vi "Panel.vi"(11 "SequenceViewPanel in":refnum<class "SequenceViewPanel.lvclass">) -> ()   [LabVIEW 2020, in "TSnax UI.lvlib" / "SequenceViewPanel.lvclass"]
uses:
  SequenceViewPanel.lvclass
  C:/Program Files (x86)/National Instruments/LabVIEW 2020/vi.lib/IlluminatedG/IG OOPanel/OOPanel/Panel/Panel.lvclass
  <vilib>/IlluminatedG/IG OOPanel/OOPanel/Panel/Basic UI State.ctl
  <vilib>/IlluminatedG/IG OOPanel/OOPanel/Panel/Panel Events.ctl
  <vilib>/IlluminatedG/IG OOPanel/OOPanel/Panel/Visbility Event Data.ctl
  <vilib>/IlluminatedG/IG OOPanel/OOPanel/Panel/Visibility State.ctl
  <vilib>/IlluminatedG/IG OOPanel/OOPanel/Panel/Close Reason.ctl
  Incoming Events.ctl
  Set SequenceFile Request.ctl
  TSnax/SequenceFile/SequenceFile.lvclass
  C:/dev/illuminated-g/tsnax/TSnax/PropertyObject/PropertyObject.lvclass
  Set SequenceFile Response.ctl
  Refresh Step Request.ctl
  TSnax/Step/Step.lvclass
  Error Response.ctl
  Step Result Request.ctl
  SequenceViewPanel.lvclass/SequenceViewPanel.ctl
  TSnax/PropertyObject/PropertyObject.lvclass/PropertyObject.ctl
  Mark Trace Data.ctl
  Trace Marker.ctl
  TSnax/Step Group.ctl
  TSnax/PropertyObject/PropertyObject Ref.vi
  UIMsg Callback.vi
  TSnax/PropertyObject/PropertyObject.lvclass
  TSnax/Sequence/Sequence.lvclass
  <vilib>/IlluminatedG/IG OOPanel/OOPanel/Panel/Panel.lvclass
  <vilib>/IlluminatedG/IG OOPanel/OOPanel/OOPanel.lvlib
  TSnax UI.lvlib
  TSnax/TSnax.lvlib
  TSnax/Engine/Engine.lvclass
  C:/dev/illuminated-g/tsnax/TSnax UI/SequenceViewPanel/SequenceViewPanel.lvclass
  C:/dev/illuminated-g/tsnax/TSnax/PropertyObjectFile/PropertyObjectFile.lvclass
  C:/dev/illuminated-g/tsnax/TSnax/SequenceFile/SequenceFile.lvclass
  TSnax/UIMessage/UIMessage.lvclass
panel:
  out "Markers":picture
  in  "Steps":string(tree)
  in  "Sequences":string(tree)
  in  "Variables":string(tree)
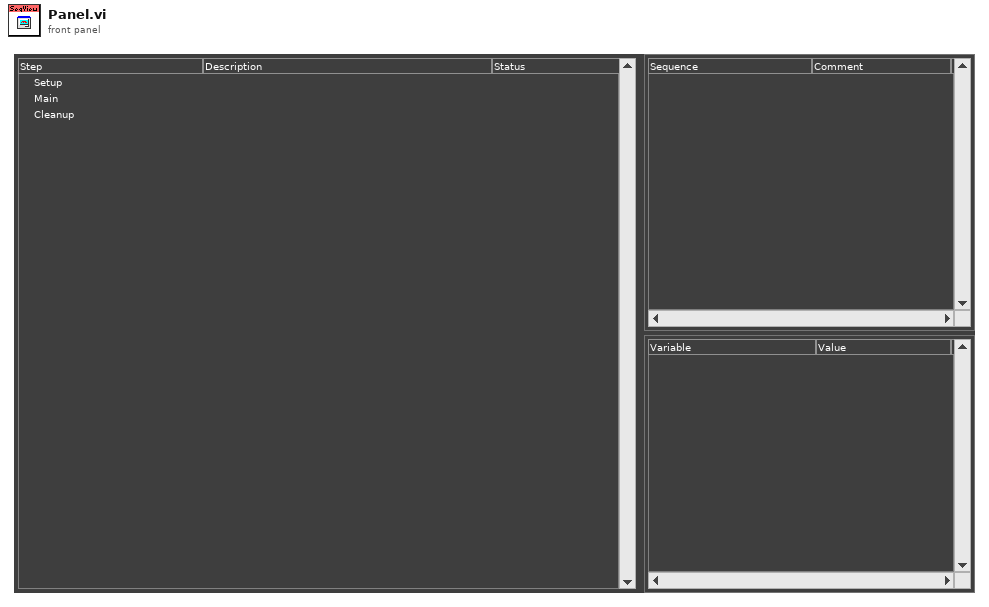
[diagram p1: front panel]
types:
  T1 = typedef "OOPanel.lvlib/Panel.lvclass/Basic UI State.ctl" = enum16{"Init", "Run", "Close"}
  T2 = typedef "TSnax UI.lvlib/SequenceViewPanel.lvclass/Set SequenceFile Response.ctl" = cluster{"Error":errorcluster}
  T3 = typedef "TSnax UI.lvlib/SequenceViewPanel.lvclass/Set SequenceFile Request.ctl" = cluster{"SequenceFile":refnum<class "SequenceFile.lvclass">, "Notifier":refnum<notifier>, "SequenceIndex":i32}
  T4 = typedef "TSnax UI.lvlib/SequenceViewPanel.lvclass/Mark Trace Data.ctl" = cluster{"Trace Marker":T5}
  T5 = typedef "TSnax UI.lvlib/SequenceViewPanel.lvclass/Trace Marker.ctl" = cluster{"TSnax:SequenceFile":refnum<class "SequenceFile.lvclass">, "SequenceIndex":i32, "StepGroup":i32, "PreviousStepIndex":i32, "NextStepIndex":i32}
  T6 = typedef "TSnax UI.lvlib/Error Response.ctl" = cluster{"Error":errorcluster}
  T7 = typedef "TSnax.lvlib/Step Group.ctl" = enum16{"Setup", "Main", "Cleanup"}
  T8 = typedef "TSnax UI.lvlib/SequenceViewPanel.lvclass/Incoming Events.ctl" = cluster{"Set SequenceFile":refnum<user-event>, "Show Sequence":refnum<user-event>, "Refresh Step":refnum<user-event>, "Step Result":refnum<user-event>}
  T9 = typedef "OOPanel.lvlib/Panel.lvclass/Panel Events.ctl" = cluster{"Visbility":refnum<user-event>, "Close":refnum<user-event>}
  T10 = cluster{"Panel":refnum<event-registration>, "Refresh Markers Reg":refnum<event-registration>, "Mark Trace Reg":refnum<event-registration>}
  T11 = typedef "OOPanel.lvlib/Visibility State.ctl" = enum16{"Idle", "Closed", "Hidden", "Visible", "Subpanel"}
  T12 = typedef "LVRectTypeDef.ctl" = cluster{"Left":i16, "Top":i16, "Right":i16, "Bottom":i16}
  T13 = typedef "LVBoundsTypeDef.ctl" = cluster{"Width":u32, "Height":u32}
  T14 = typedef "LVPoint32TypeDef.ctl" = cluster{"Horizontal":i32, "Vertical":i32}
  T15 = typedef "LVNodeAndColumnTypeDef.ctl" = cluster{"Node":string, "Column":i32}
  T16 = typedef "TSnax UI.lvlib/SequenceViewPanel.lvclass/Ref Data.ctl" = cluster{"Insert Line":i32, "SequenceFile":refnum<class "SequenceFile.lvclass">, "Sequence":string, "Trace Marker":i32, "Execution":refnum<class "Execution.lvclass">}
  T17 = typedef "TSnax.lvlib/UIMsg.ctl" = enum16{"Unknown", "BreakOnUserRequest", "BreakOnBreakpoint", "BreakOnRunTimeError", "Trace", "TerminatingExecution", "AbortingExecution", "KillingExecutionThreads", "EndExecution", "ShutDownComplete", "StartExecution", "ProgressPercent", "ProgressText", "StartInteractiveExecution", "EndInteractiveExecution", "TerminatingInteractiveExecution", "TerminationCancelled", "ResumeFromBreak", "StartFileExecution", "EndFileExecution", "ShutDownCancelled", "LocalizationSettingChanged", "OpenWindows", "TileWindows", "CascadeWindows", "ReportChanged", "CloseWindows", "RefreshWindows", "ClientFileChanged", "DisplayReport", "ModelState_Initializing", "ModelState_Waiting", "ModelState_Identified", "ModelState_BeginTesting", "ModelState_TestingComplete", "ModelState_PostProcessingComplete", "ModelState_EnabledStateSet", "ReportLocationChanged", "GotoLocation", "PushUndoItem", "OutputMessages", "TypePaletteFileListChanged", "NonTerminatingThreadsArePreventingTermination", "ModelState_PostProcessing", "ReportCollectionChanged", "RuntimeError"}
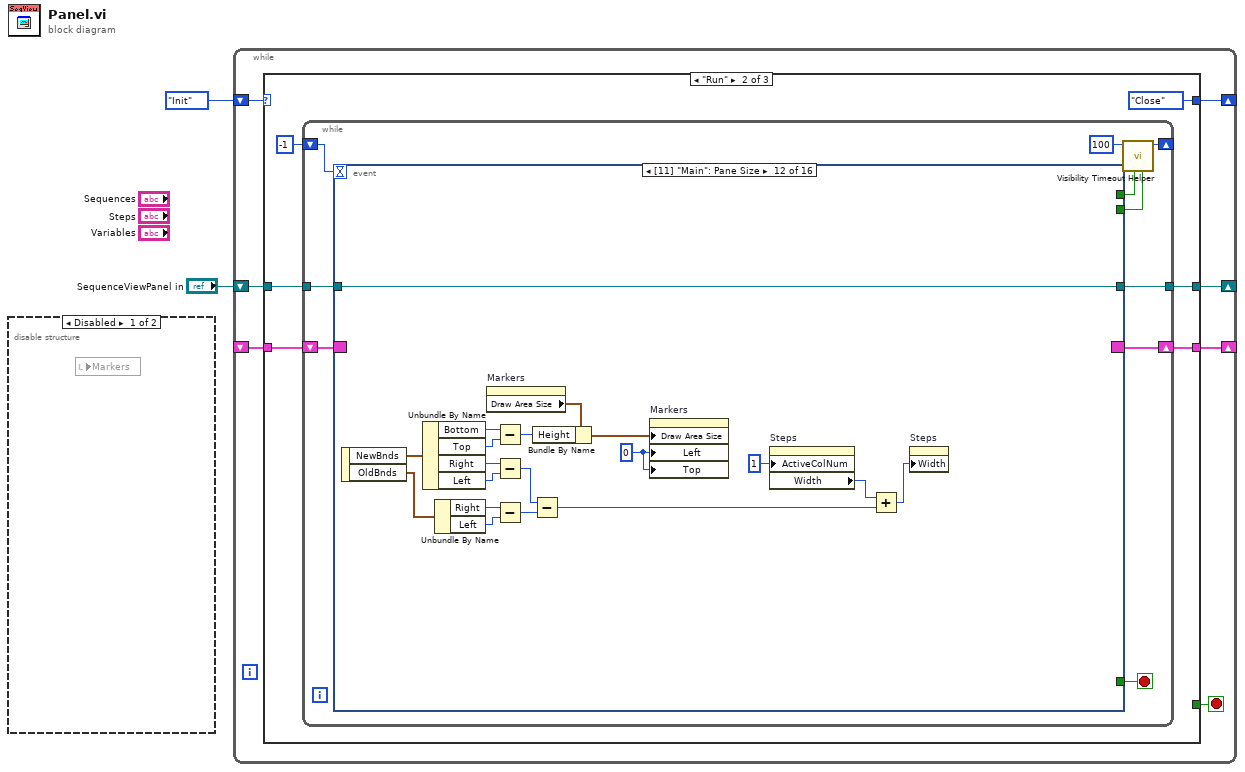
[diagram p0: block diagram]
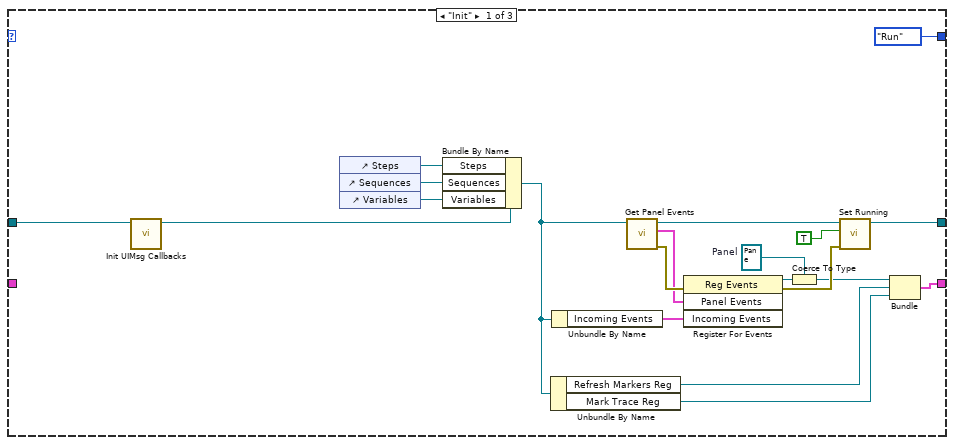
[diagram p3: hidden frame]
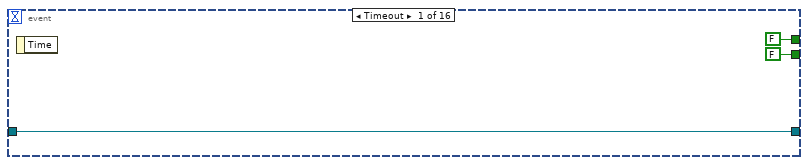
[diagram p4: hidden frame]
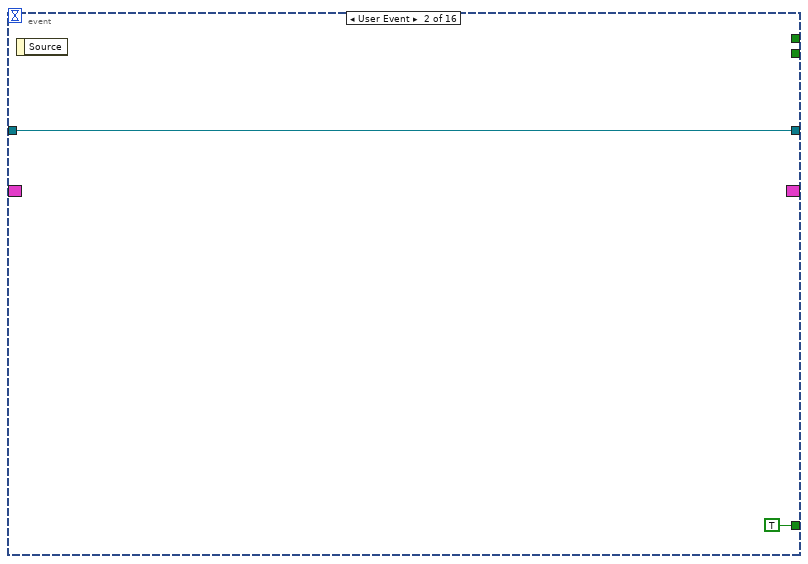
[diagram p5: hidden frame]
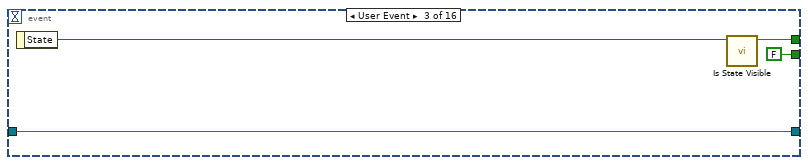
[diagram p6: hidden frame]
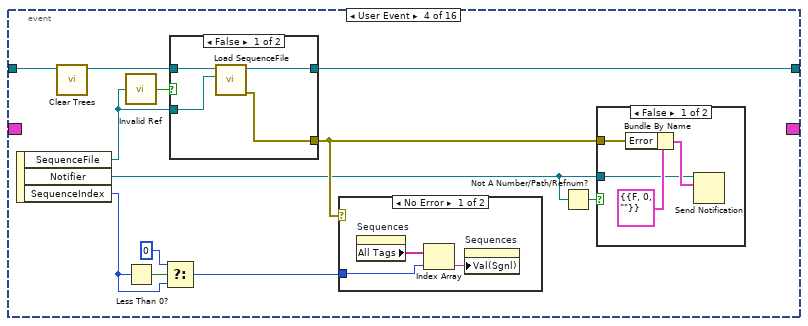
[diagram p7: hidden frame]
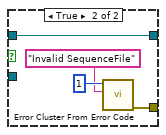
[diagram p10: hidden frame]
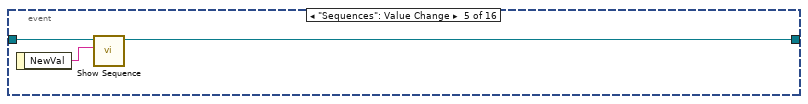
[diagram p11: hidden frame]
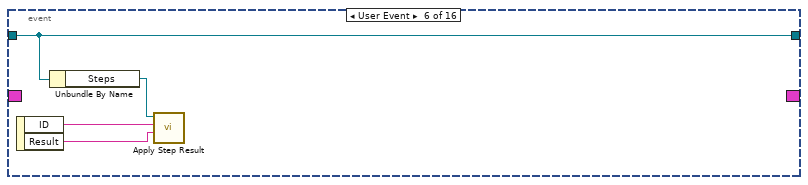
[diagram p12: hidden frame]
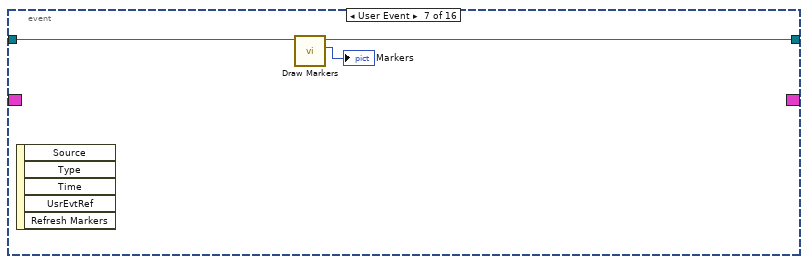
[diagram p13: hidden frame]
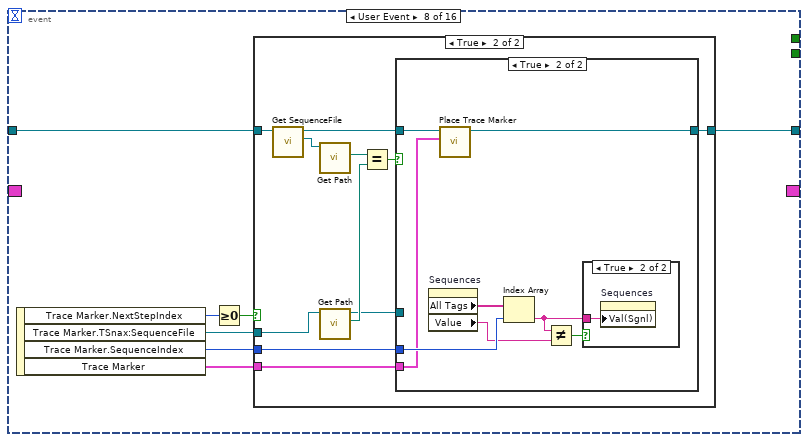
[diagram p14: hidden frame]
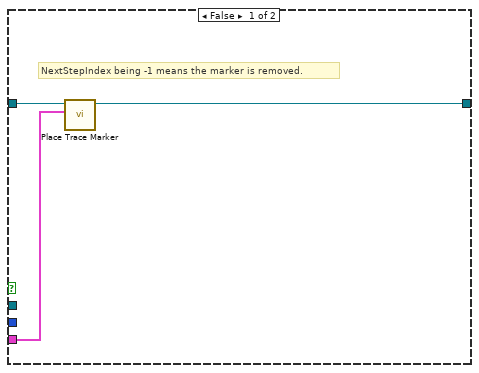
[diagram p15: hidden frame]
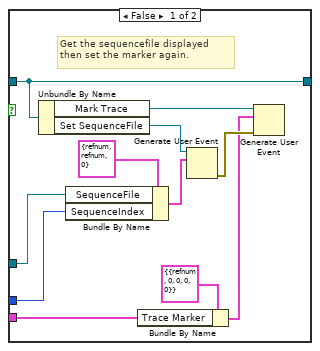
[diagram p16: hidden frame]
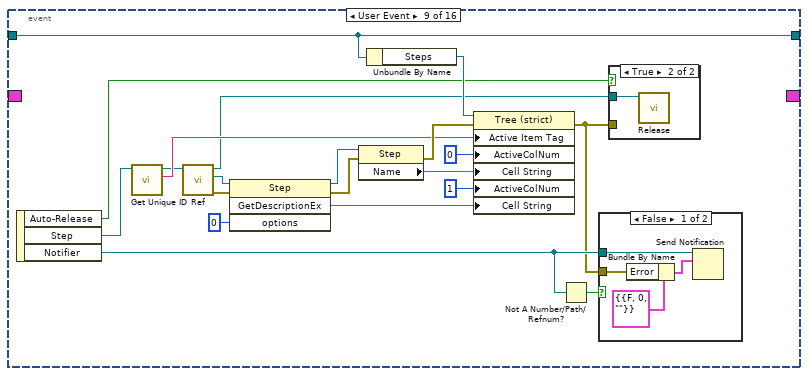
[diagram p18: hidden frame]
diagram:
  n1 = disable-structure shown="Disabled" {
    frame Disabled {
      n2 = local read "Markers"() -> ()  [unwired: 1 in]
    }
    frame Enabled {
    }
  }
  n3 = while {
    shift-right: [w8] -> _
    shift-left: _ -> [w9]
    shift-right: [w6] -> _
    shift-left: Basic_UI_State."Init" ("Basic UI State") -> [w7]
    shift-right: [w4] -> _
    shift-left: "SequenceViewPanel in" -> [w3]
    stop <- w5 stop-if-true
    n4 = case shown="\"Run\"" w7 {
      tunnel: w9 -> [_ w35 w252]
      tunnel: [w16 w33 _] -> w8
      tunnel: [Basic_UI_State."Run" ("Basic UI State") Basic_UI_State."Close" ("Basic UI State") Basic_UI_State."Close" ("Basic UI State")] -> w6
      tunnel: [_ _ TRUE] -> w5
      tunnel: [w12 w30 w251] -> w4
      tunnel: w3 -> [w11 w31 w250]
      frame "Init" {
        w14 = refnum<event-registration> refnum  # Panel
        n5 = call "Init UIMsg Callbacks.vi"("SequenceViewPanel in"=w11) -> ("SequenceViewPanel out"=w10:refnum<class "SequenceViewPanel.lvclass">)  [unwired: 9 in, 1 out]
        n6 = control-ref of="Steps"() -> (w23:refnum<vi>)
        n7 = control-ref of="Sequences"() -> (w22:refnum<vi>)
        n8 = control-ref of="Variables"() -> (w21:refnum<vi>)
        n9 = Bundle By Name(cluster=w10, "Steps"=w23, "Sequences"=w22, "Variables"=w21) -> (w18:refnum<class "SequenceViewPanel.lvclass">)
        n10 = Unbundle By Name(w18) -> ("Refresh Markers Reg"=w17:refnum<event-registration>, "Mark Trace Reg"=w13:refnum<event-registration>)
        n11 = Unbundle By Name(w18) -> ("Incoming Events"=w24:T8)
        n12 = call <vilib>:"Get Panel Events.vi"("Panel in"=w18) -> ("error out"=w29:errorcluster, "Panel Events"=w26:T9, "Panel out"=w20:refnum<class "SequenceViewPanel.lvclass">)  [unwired: 8 in]
        n13 = register-events(error in=w29, w26, w24) -> (reference out=w19:refnum<event-registration>, error out=w27:errorcluster)  [unwired: 1 in]
        n14 = Coerce To Type(0:w19, 1:w14) -> (2:w15:refnum<event-registration>)
        n15 = call <vilib>:"Set Running.vi"("error in (no error)"=w27, "Running"=TRUE, "Panel in"=w20) -> ("Panel out"=w12:refnum<class "SequenceViewPanel.lvclass">)  [unwired: 7 in, 1 out]
        n16 = Bundle("Panel"=w15, "Refresh Markers Reg"=w17, "Mark Trace Reg"=w13) -> (w16:T10)  [unwired: 1 in]
      }
      frame "Run" {
        n17 = while {
          shift-right: [w41] -> w33
          shift-left: w35 -> [w42]
          shift-right: [w44] -> _
          shift-left: -1 ("Timeout") -> [w43]
          tunnel: w31 -> [w37]
          tunnel: [w36] -> w30
          stop <- w38 stop-if-true
          n18 = event shown="[11] \"Main\": Pane Size" {
            selector: w42 -> [_ _ _ _ _ _ _ _ _ _ _ _ _ _ _ _]
            dyn-events: [_ _ _ _ _ _ _ _ _ _ _ _ _ _ _ _] -> w41
            timeout: w43 -> [_ _ _ _ _ _ _ _ _ _ _ _ _ _ _ _]
            tunnel: [FALSE _ w53 _ _ _ _ _ _ _ _ _ _ _ _ _] -> w40
            tunnel: [FALSE _ FALSE _ _ _ _ _ _ _ _ _ _ _ _ _] -> w39
            tunnel: [_ TRUE _ _ _ _ _ _ _ _ _ _ _ _ _ _] -> w38
            tunnel: w37 -> [w46 w49 w51 w66 w84 w88 w91 w98 w150 w164 w188 w207 w212 w213 w222 w241]
            tunnel: [w46 w49 w51 w63 w82 w88 w90 w96 w150 w159 w188 w207 w209 w213 w216 w240] -> w36
            event Timeout {
              n19 = event-data() -> ()  [unwired: 1 in, 1 out]
            }
            event User Event {
              n20 = event-data() -> ()  [unwired: 1 in, 1 out]
            }
            event User Event {
              n21 = event-data() -> ("State"=w54:T11)  [unwired: 1 in]
              n22 = call <vilib>:"Is State Visible.vi"("Visibility"=w54) -> ("Visible"=w53:bool)  [unwired: 10 in]
            }
            event User Event {
              n23 = event-data() -> ("SequenceFile"=w62:refnum<class "SequenceFile.lvclass">, "Notifier"=w56:refnum<notifier>, "SequenceIndex"=w59:i32)  [unwired: 1 in]
              n24 = call "Clear Trees.vi"("SequenceViewPanel in"=w66) -> ("SequenceViewPanel out"=w64:refnum<class "SequenceViewPanel.lvclass">)  [unwired: 9 in, 1 out]
              n25 = call "Invalid Ref.vi"("PropertyObject"=w62) -> ("Not a Valid Ref?"=w65:bool)
              n26 = Less Than 0?(x=w59) -> (x < 0?=w60:bool)
              n27 = Select(t=0, s=w60, f=w59) -> (s? t:f=w57:i32)
              n28 = case shown="False" w65 {
                tunnel: w64 -> [w77 w81]
                tunnel: [w75 w81] -> w63
                tunnel: w62 -> [w76 _]
                tunnel: [w74 w78] -> w61
                frame False {
                  n29 = call "Load SequenceFile.vi"("SequenceFile"=w76, "SequenceViewPanel in"=w77) -> ("error out"=w74:errorcluster, "SequenceViewPanel out"=w75:refnum<class "SequenceViewPanel.lvclass">)  [unwired: 8 in]
                }
                frame True {
                  n30 = call <vilib>:"Error Cluster From Error Code.vi"("error message (\"\")"="Invalid SequenceFile" ("error message (\"\")"), "error code (0)"=1) -> ("error out"=w78:errorcluster)  [unwired: 7 in]
                }
              }
              n31 = case shown="No Error" w61 {
                tunnel: w57 -> [w71 _]
                frame No Error {
                  n32 = property on="Sequences" class="Tree (strict)"() -> ("All Tags"=w73:string[])  [unwired: 2 in, 2 out]
                  n33 = Index Array(array=w73, index=w71) -> (element=w72:string)
                  n34 = property on="Sequences" class="Tree (strict)"("Val(Sgnl)"=w72) -> ()  [unwired: 2 in, 2 out]
                }
                frame Error {
                }
              }
              n35 = Not A Number/Path/Refnum?(number/path/refnum=w56) -> (NaN/Path/Refnum?=w55:bool)
              n36 = case shown="False" w55 {
                tunnel: w61 -> [w68 _]
                tunnel: w56 -> [w67 _]
                frame False {
                  n37 = Bundle By Name(cluster=T2 {"Error"={"status"=FALSE, "code"=0, "source"=""}} ("notification"), "Error"=w68) -> (w69:T2)
                  n38 = Send Notification(notification=w69, notifier=w67) -> ()  [unwired: 1 in, 2 out]
                }
                frame True {
                }
              }
            }
            event "Sequences": Value Change {
              n39 = event-data() -> ("NewVal"=w83:string)  [unwired: 1 in]
              n40 = call "Show Sequence.vi"("Sequence"=w83, "SequenceViewPanel in"=w84) -> ("SequenceViewPanel out"=w82:refnum<class "SequenceViewPanel.lvclass">)  [unwired: 8 in, 1 out]
            }
            event User Event {
              n41 = event-data() -> ("ID"=w86:string, "Result"=w85:string)  [unwired: 1 in]
              n42 = Unbundle By Name(w88) -> ("Steps"=w87:refnum<vi>)
              n43 = call "Apply Step Result.vi"("ResultStatus"=w85, "UniqueStepId"=w86, "Steps Tree In"=w87) -> ()  [unwired: 7 in, 2 out]
            }
            event User Event {
              n44 = event-data() -> ()  [unwired: 1 in, 5 out]
              n45 = call "Draw Markers.vi"("SequenceViewPanel in"=w91) -> ("Markers"=→"Markers":picture, "SequenceViewPanel out"=w90:refnum<class "SequenceViewPanel.lvclass">)  [unwired: 8 in, 1 out]
            }
            event User Event {
              n46 = event-data() -> ("Trace Marker.NextStepIndex"=w93:i32, "Trace Marker.TSnax:SequenceFile"=w94:refnum<class "SequenceFile.lvclass">, "Trace Marker.SequenceIndex"=w95:i32, "Trace Marker"=w97:T5)  [unwired: 1 in]
              n47 = Greater Or Equal To 0?(x=w93) -> (x >= 0?=w92:bool)
              n48 = case shown="True" w92 {
                tunnel: w98 -> [w101 w112]
                tunnel: w97 -> [w100 w111]
                tunnel: [w99 w108] -> w96
                tunnel: w95 -> [_ w107]
                tunnel: w94 -> [_ w103]
                frame False {
                  # "NextStepIndex being -1 means the marker is removed."
                  n49 = call "Place Trace Marker.vi"("Trace Marker"=w100, "SequenceViewPanel in"=w101) -> ("SequenceViewPanel out"=w99:refnum<class "SequenceViewPanel.lvclass">)  [unwired: 8 in, 1 out]
                }
                frame True {
                  n50 = call "Get SequenceFile.vi"("SequenceViewPanel in"=w112) -> ("SequenceFile"=w106:refnum<class "SequenceFile.lvclass">, "SequenceViewPanel out"=w109:refnum<class "SequenceViewPanel.lvclass">)  [unwired: 8 in, 1 out]
                  n51 = call-dynamic "Get Path.vi"("SequenceFile in"=w106) -> ("Path"=w105:path)  [unwired: 8 in, 2 out]
                  n52 = call-dynamic "Get Path.vi"("SequenceFile in"=w103) -> ("Path"=w104:path, "SequenceFile out"=w102:refnum<class "SequenceFile.lvclass">)  [unwired: 8 in, 1 out]
                  n53 = Equal?(x=w105, y=w104) -> (x = y?=w110:bool)
                  n54 = case shown="True" w110 {
                    tunnel: w111 -> [w119 w124]
                    tunnel: w109 -> [w118 w126]
                    tunnel: w102 -> [w114 _]
                    tunnel: [w118 w125] -> w108
                    tunnel: w107 -> [w113 w130]
                    frame False {
                      # "Get the sequencefile displayed then set the marker again."
                      n55 = Unbundle By Name(w118) -> ("Mark Trace"=w122:refnum<user-event>, "Set SequenceFile"=w117:refnum<user-event>)
                      n56 = Bundle By Name(cluster=T3 {"SequenceFile"=refnum, "Notifier"=refnum, "SequenceIndex"=0} ("event data"), "SequenceFile"=w114, "SequenceIndex"=w113) -> (w115:T3)
                      n57 = Bundle By Name(cluster=T4 {"Trace Marker"={"TSnax:SequenceFile"=refnum, "SequenceIndex"=0, "StepGroup"=0, "PreviousStepIndex"=0, "NextStepIndex"=0}} ("event data"), "Trace Marker"=w119) -> (w120:T4)
                      n58 = Generate User Event(user event=w117, event data cluster=w115) -> (error out=w123:errorcluster)  [unwired: 2 in, 1 out]
                      n59 = Generate User Event(user event=w122, event data cluster=w120, error in=w123) -> ()  [unwired: 1 in, 2 out]
                    }
                    frame True {
                      n60 = property on="Sequences" class="Tree (strict)"() -> ("All Tags"=w131:string[], "Value"=w129:string)  [unwired: 2 in, 2 out]
                      n61 = call "Place Trace Marker.vi"("Trace Marker"=w124, "SequenceViewPanel in"=w126) -> ("SequenceViewPanel out"=w125:refnum<class "SequenceViewPanel.lvclass">)  [unwired: 8 in, 1 out]
                      n62 = Index Array(array=w131, index=w130) -> (element=w128:string)
                      n63 = Not Equal?(x=w128, y=w129) -> (x != y?=w127:bool)
                      n64 = case shown="True" w127 {
                        tunnel: w128 -> [_ w132]
                        frame False {
                        }
                        frame True {
                          n65 = property on="Sequences" class="Tree (strict)"("Val(Sgnl)"=w132) -> ()  [unwired: 2 in, 2 out]
                        }
                      }
                    }
                  }
                }
              }
            }
            event User Event {
              n66 = event-data() -> ("Auto-Release"=w133:bool, "Step"=w151:refnum<class "Step.lvclass">, "Notifier"=w137:refnum<notifier>)  [unwired: 1 in]
              n67 = call "Get Unique ID.vi"("Step in"=w151) -> ("Unique ID"=w148:string, "Step out"=w147:refnum<class "Step.lvclass">)  [unwired: 8 in, 1 out]
              n68 = call "Ref.vi"("Step in"=w147) -> ("error out"=w145:errorcluster, "Step"=w146:refnum<k7>, "Step out"=w135:refnum<class "Step.lvclass">)  [unwired: 8 in]
              n69 = invoke class="Step" method="GetDescriptionEx"(reference=w146, error in=w145, "options"=0) -> (reference out=w140:refnum<k7>, error out=w139:errorcluster, "GetDescriptionEx"=w142:string)  [unwired: 1 in, 1 out]
              n70 = property class="Step"(reference=w140, error in=w139) -> (error out=w152:errorcluster, "Name"=w138:string)  [unwired: 1 out]
              n71 = Unbundle By Name(w150) -> ("Steps"=w149:refnum<vi>)
              n72 = property class="Tree (strict)"(reference=w149, error in=w152, "Active Item Tag"=w148, "ActiveColNum"=0 ("Active Cell:Active Column Number"), "Cell String"=w138, "ActiveColNum"=1 ("Active Cell:Active Column Number"), "Cell String"=w142) -> (error out=w134:errorcluster)  [unwired: 1 out]
              n73 = Not A Number/Path/Refnum?(number/path/refnum=w137) -> (NaN/Path/Refnum?=w136:bool)
              n74 = case shown="False" w136 {
                tunnel: w134 -> [w155 _]
                tunnel: w137 -> [w154 _]
                frame False {
                  n75 = Bundle By Name(cluster=T6 {"Error"={"status"=FALSE, "code"=0, "source"=""}} ("notification"), "Error"=w155) -> (w156:T6)
                  n76 = Send Notification(notification=w156, notifier=w154) -> ()  [unwired: 1 in, 2 out]
                }
                frame True {
                }
              }
              n77 = case shown="True" w133 {
                tunnel: w135 -> [_ w153]
                tunnel: w134 -> [_ _]
                frame False {
                }
                frame True {
                  n78 = call-dynamic "Release.vi"("Step in"=w153) -> ()  [unwired: 10 in, 1 out]
                }
              }
            }
            event "Steps": Double Click {
              n79 = event-data() -> ("Tag"=w158:string)  [unwired: 1 in]
              n80 = call "Get Displayed Sequence.vi"("SequenceViewPanel in"=w164) -> ("Sequence"=w161:string, "SequenceViewPanel out"=w163:refnum<class "SequenceViewPanel.lvclass">)  [unwired: 8 in, 1 out]
              n81 = call "Get SequenceFile.vi"("SequenceViewPanel in"=w163) -> ("SequenceFile"=w162:refnum<class "SequenceFile.lvclass">, "SequenceViewPanel out"=w160:refnum<class "SequenceViewPanel.lvclass">)  [unwired: 8 in, 1 out]
              n82 = Scan From String(input string=w158, default 1=Step_Group."Setup" ("Step Group")) -> (error out=w165:errorcluster)  [unwired: 4 in, 2 out]
              n83 = case shown="Error .." w165 {
                tunnel: w162 -> [_ w178]
                tunnel: w161 -> [_ w177]
                tunnel: w160 -> [w167 w171]
                tunnel: [w167 w169] -> w159
                tunnel: w158 -> [_ w175]
                frame No Error {
                  # "Is a group listing, don't need to try and open edit."
                }
                frame Error {
                  n84 = call "Sequence by Name.vi"("Sequence Name"=w177, "SequenceFile in"=w178) -> ("error out"=w179:errorcluster, "Sequence"=w176:refnum<class "Sequence.lvclass">)  [unwired: 7 in, 1 out]
                  n85 = call "Step by Name or ID.vi"("error in (no error)"=w179, "Name or ID"=w175, "Sequence in"=w176) -> ("error out"=w173:errorcluster, "Step"=w172:refnum<class "Step.lvclass">, "Sequence out"=w174:refnum<class "Sequence.lvclass">)  [unwired: 6 in]
                  n86 = call-dynamic "Release.vi"("error in (no error)"=w173, "Sequence in"=w174) -> ()  [unwired: 9 in, 1 out]
                  n87 = call "Run Edit.vi"("error in (no error)"=w173, "Step in"=w172) -> ("error out"=w168:errorcluster, "Step out"=w170:refnum<class "Step.lvclass">)  [unwired: 7 in, 1 out]
                  n88 = call <vilib>:"Simple Error Handler.vi"("error in (no error)"=w168) -> ()  [unwired: 4 in, 5 out]
                  n89 = case shown="No Error" w168 {
                    tunnel: w171 -> [w183 w184]
                    tunnel: w170 -> [w182 _]
                    tunnel: [w180 w184] -> w169
                    frame No Error {
                      n90 = call "Refresh Step.vi"("Skip Response? (F)"=TRUE, "Step"=w182, "SequenceViewPanel in"=w183) -> ("SequenceViewPanel out"=w180:refnum<class "SequenceViewPanel.lvclass">)  [unwired: 7 in, 1 out]
                    }
                    frame Error {
                    }
                  }
                }
              }
            }
            event "Steps": event type 3.0.x80000011; "Steps": Item Open? {
              # "Don't want default behavior of double-clicking parent items to cause collapse/expand."
              n91 = event-data() -> ("Tag"=w186:string)  [unwired: 1 in, 4 out]
              n92 = invoke on="Steps" class="Tree (strict)" method="Double Click"() -> ("Double Click"=w187:string)  [unwired: 3 in, 2 out]
              n93 = Equal?(x=w187, y=w186) -> (x = y?=w185:bool)
              n94 = event-data("Discard?"=w185) -> ()  [unwired: 1 in, 1 out]
            }
            event Pane Size {
              w200 = 0 ("Position:Left")
              n95 = event-data() -> ("NewBnds"=w204:T12, "OldBnds"=w198:T12)  [unwired: 1 in]
              n96 = Unbundle By Name(w204) -> ("Bottom"=w203:i16, "Top"=w202:i16, "Right"=w195:i16, "Left"=w194:i16)
              n97 = Unbundle By Name(w198) -> ("Right"=w197:i16, "Left"=w196:i16)
              n98 = property on="Markers" class="Pict"() -> ("Draw Area Size"=w205:T13)  [unwired: 2 in, 2 out]
              n99 = Subtract(x=w203, y=w202) -> (x-y=w201:i16)
              n100 = Subtract(x=w195, y=w194) -> (x-y=w192:i16)
              n101 = Subtract(x=w197, y=w196) -> (x-y=w193:i16)
              n102 = Subtract(x=w192, y=w193) -> (x-y=w191:i16)
              n103 = Bundle By Name(cluster=w205, "Height"=w201) -> (w206:T13)
              n104 = property on="Markers" class="Pict"("Draw Area Size"=w206, "Left"=w200, "Top"=w200) -> ()  [unwired: 2 in, 2 out]
              n105 = property on="Steps" class="Tree (strict)"("ActiveColNum"=1 ("Active Cell:Active Column Number")) -> ("Width"=w190:i32)  [unwired: 2 in, 2 out]
              n106 = Add(x=w190, y=w191) -> (x+y=w189:i32)
              n107 = property on="Steps" class="Tree (strict)"("Width"=w189) -> ()  [unwired: 2 in, 2 out]
            }
            event "Steps": event type 3.0.xa000003a; "Steps": Drag Enter {
              n108 = event-data() -> ("Coords"=w211:T14, "Available Data Names"=w210:string[])  [unwired: 1 in, 7 out]
              n109 = call "Handle Drag.vi"("Available Data Names"=w210, "Coords"=w211, "SequenceViewPanel in"=w212) -> ("SequenceViewPanel out"=w209:refnum<class "SequenceViewPanel.lvclass">, "Accepted?"=w208:bool)  [unwired: 4 in, 3 out]
              n110 = event-data("Accepted?"=w208) -> ()  [unwired: 1 in, 1 out]
            }
            event "Steps": Drag Starting? {
              n111 = event-data() -> ()  [unwired: 1 in, 10 out]
              n112 = event-data() -> ()  [unwired: 4 in, 1 out]
            }
            event "Steps": Drop {
              n113 = event-data() -> ("Coords"=w229:T14, "Available Data Names"=w228:string[])  [unwired: 1 in, 7 out]
              n114 = Unbundle By Name(w222) -> ("Steps"=w221:refnum<vi>)
              n115 = property class="Tree (strict)"(reference=w221) -> (reference out=w220:refnum<vi>, error out=w218:errorcluster, "TopLeft"=w215:T15)  [unwired: 1 in]
              n116 = call "Handle Drag.vi"("Done? (F)"=TRUE, "Available Data Names"=w228, "Coords"=w229, "SequenceViewPanel in"=w222) -> ("Tag"=w226:string, "Step Type Name"=w224:string, "SequenceViewPanel out"=w227:refnum<class "SequenceViewPanel.lvclass">, "Accepted?"=w225:bool, "Index"=w214:i32)  [unwired: 3 in]
              n117 = call "Drop Step by Type.vi"("Index"=w214, "Tag"=w226, "Step Type Name"=w224, "SequenceViewPanel in"=w227) -> ("error out"=w217:errorcluster, "SequenceViewPanel out"=w223:refnum<class "SequenceViewPanel.lvclass">)  [unwired: 6 in]
              n118 = call <vilib>:"Simple Error Handler.vi"("error in (no error)"=w217) -> ()  [unwired: 4 in, 5 out]
              n119 = case shown="No Error" w217 {
                selector: w217 -> [_ w239]
                tunnel: w223 -> [w237 w238]
                tunnel: [w234 w239] -> w219
                tunnel: w218 -> [w233 _]
                tunnel: [w231 w238] -> w216
                frame No Error {
                  n120 = call "Get Displayed Sequence.vi"("error in (no error)"=w233, "SequenceViewPanel in"=w237) -> ("error out"=w232:errorcluster, "Sequence"=w235:string, "SequenceViewPanel out"=w236:refnum<class "SequenceViewPanel.lvclass">)  [unwired: 7 in]
                  n121 = call "Show Sequence.vi"("error in (no error)"=w232, "Sequence"=w235, "SequenceViewPanel in"=w236) -> ("error out"=w234:errorcluster, "SequenceViewPanel out"=w231:refnum<class "SequenceViewPanel.lvclass">)  [unwired: 7 in]
                }
                frame Error {
                }
              }
              n122 = property class="Tree (strict)"(reference=w220, error in=w219, "TopLeft"=w215) -> ()  [unwired: 2 out]
              n123 = event-data("Accepted?"=w225) -> ()  [unwired: 1 in, 1 out]
            }
            event "Steps": Mouse Up {
              n124 = event-data() -> ()  [unwired: 1 in, 8 out]
              n125 = Unbundle By Name(w241) -> ("Ref"=w242:refnum<data-value>)
              n126 = in-place {
                n127 = in-place-dvr #1(w242) -> (w245:T16)  [unwired: 1 out]
                n128 = Bundle By Name(cluster=w245, "Insert Line"=-1 ("Insert Index")) -> (w244:T16)
                n129 = in-place-dvr #1(w244) -> ()  [unwired: 2 out]
              }
              n130 = call "Fire Refresh Markers.vi"("SequenceViewPanel in"=w241) -> ("SequenceViewPanel out"=w240:refnum<class "SequenceViewPanel.lvclass">)  [unwired: 9 in, 1 out]
            }
          }
          n131 = call <vilib>:"Visibility Timeout Helper.vi"("Update?"=w39, "Use Timeout?"=w40, "Visible Timeout mS"=100) -> ("Timeout"=w44:i32)  [unwired: 8 in]
        }
      }
      frame "Close" {
        n132 = Unregister For Events(event registration refnum=w252) -> (error out=w254:errorcluster)  [unwired: 1 in]
        n133 = Unbundle By Name(w250) -> ("Engine"=w249:refnum<class "Engine.lvclass">, "UIMsg Callback ID"=w248:i32)
        n134 = vi-ref "TSnax UI.lvlib:SequenceViewPanel.lvclass:UIMsg Callback.vi"() -> (w247:refnum<vi>)
        n135 = call "Registered UIMsg Codes.vi"() -> ("UIMessage IDs"=w246:T17[])  [unwired: 11 in]
        n136 = call "Unregister UIMessage Callback.vi"("UIMessage IDs"=w246, "Callback ID"=w248, "Callback"=w247, "Engine in"=w249) -> ()  [unwired: 6 in, 2 out]
        n137 = call <vilib>:"Set Running.vi"("error in (no error)"=w254, "Running"=FALSE, "Panel in"=w250) -> ("Panel out"=w251:refnum<class "SequenceViewPanel.lvclass">)  [unwired: 7 in, 1 out]
      }
    }
  }
